vi "Process.vi"(8 "error in":errorcluster, 11 "Pump":refnum<class "Pump.lvclass">) -> (0 "error out":errorcluster, 3 "Pump out":refnum<class "Pump.lvclass">)   [LabVIEW 2014, in "Pump.lvclass"]
doc: "JKI State Machine Objects (SMO) 1.4.0.57\nJKI - JKI\nCopyright (c) 2018, JKI"
uses:
  Pump.lvclass
  <vilib>/JKI/JKI SMO/SMO/Typedefs/Parent Call--Enum.ctl
  Pump.lvclass/Pump.ctl
  Pump State - cluster.ctl
  <vilib>/addons/control/pid/pid.llb/PID Advanced (DBL).vi
  <vilib>/JKI/JKI SMO/SMO/SMO.lvclass
  <vilib>/addons/control/pid/NI_PID_pid.lvlib
panel:
  out "Pump State":T1(graph)
  # "For instructions on how to use the JKI State Machine Objects, examples and video tutorials, visit:\nhttp://jki.net/state-machine-objects/\n\nJKI State Machine Objects™\nhttp://jki.net/state-machine-objects/\nCopyright (C) 2005-2015, JKI <info@jki.net>\nALL RIGHTS RESERVED"
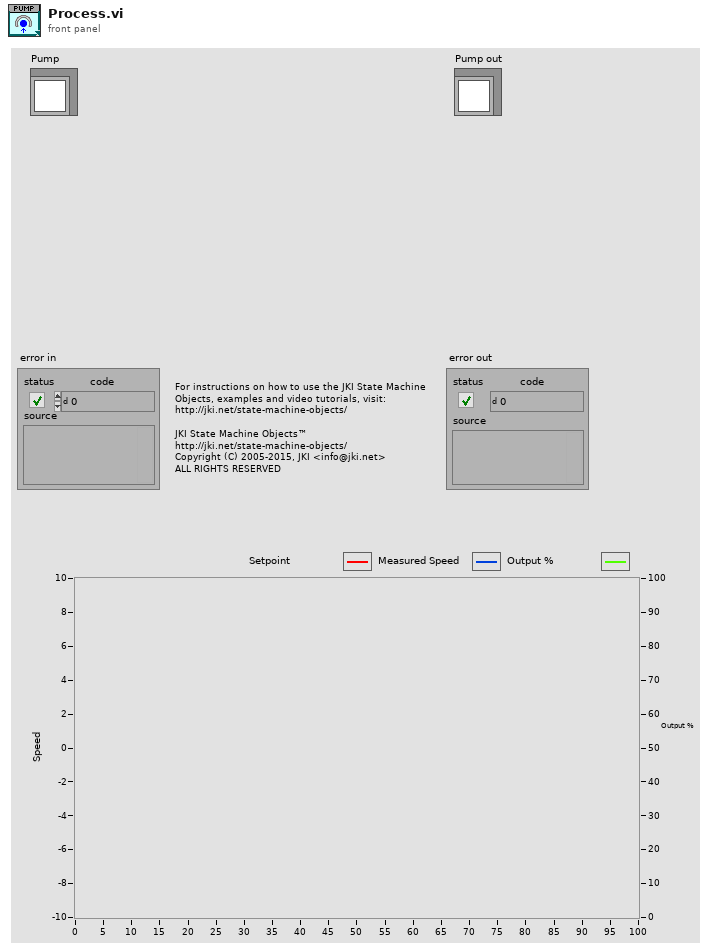
[diagram p1: front panel]
types:
  T1 = typedef "Pump.lvclass/Pump State - cluster.ctl" = cluster{"Pump Setpoint":dbl, "Pump Speed":dbl, "Output %":dbl}
  T2 = typedef "SMO.lvclass/Parent Call--Enum.ctl" = enum16{"Allows parent to run", "Does not request parent to run"}
  T3 = enum32{"invalid app kind", "Development System", "Run Time System", "Student Edition", "Embedded LabVIEW", "Evaluation", "Custom"}
  T4 = enum32{"Invalid", "Standard", "Closed", "Hidden", "Minimized", "Maximized"}
  T5 = cluster{"proportional gain (Kc)":dbl, "integral time (Ti, min)":dbl, "derivative time (Td, min)":dbl}
  T6 = typedef "Pump.lvclass/Parameters - cluster.ctl" = cluster{"Kc":dbl, "Ti":dbl, "Td":dbl, "Min Speed":dbl, "Max Speed":dbl}
  T7 = cluster{"Core":cluster{"Current VI Reference":refnum<vi>, "Close Panel on Exit?":bool, "error":errorcluster}, "Self Reference":refnum<class "Pump.lvclass">, "Parameters":T6, "Speed":dbl}
  T8 = cluster{"Current VI Reference":refnum<vi>, "Close Panel on Exit?":bool, "error":errorcluster}
  T9 = typedef "SMO.lvclass/Protected Events.ctl" = cluster{"StopProcesses":refnum<user-event>, "AbortProcesses":refnum<user-event>, "Config Changed":refnum<user-event>, "Dependency":refnum<user-event>}
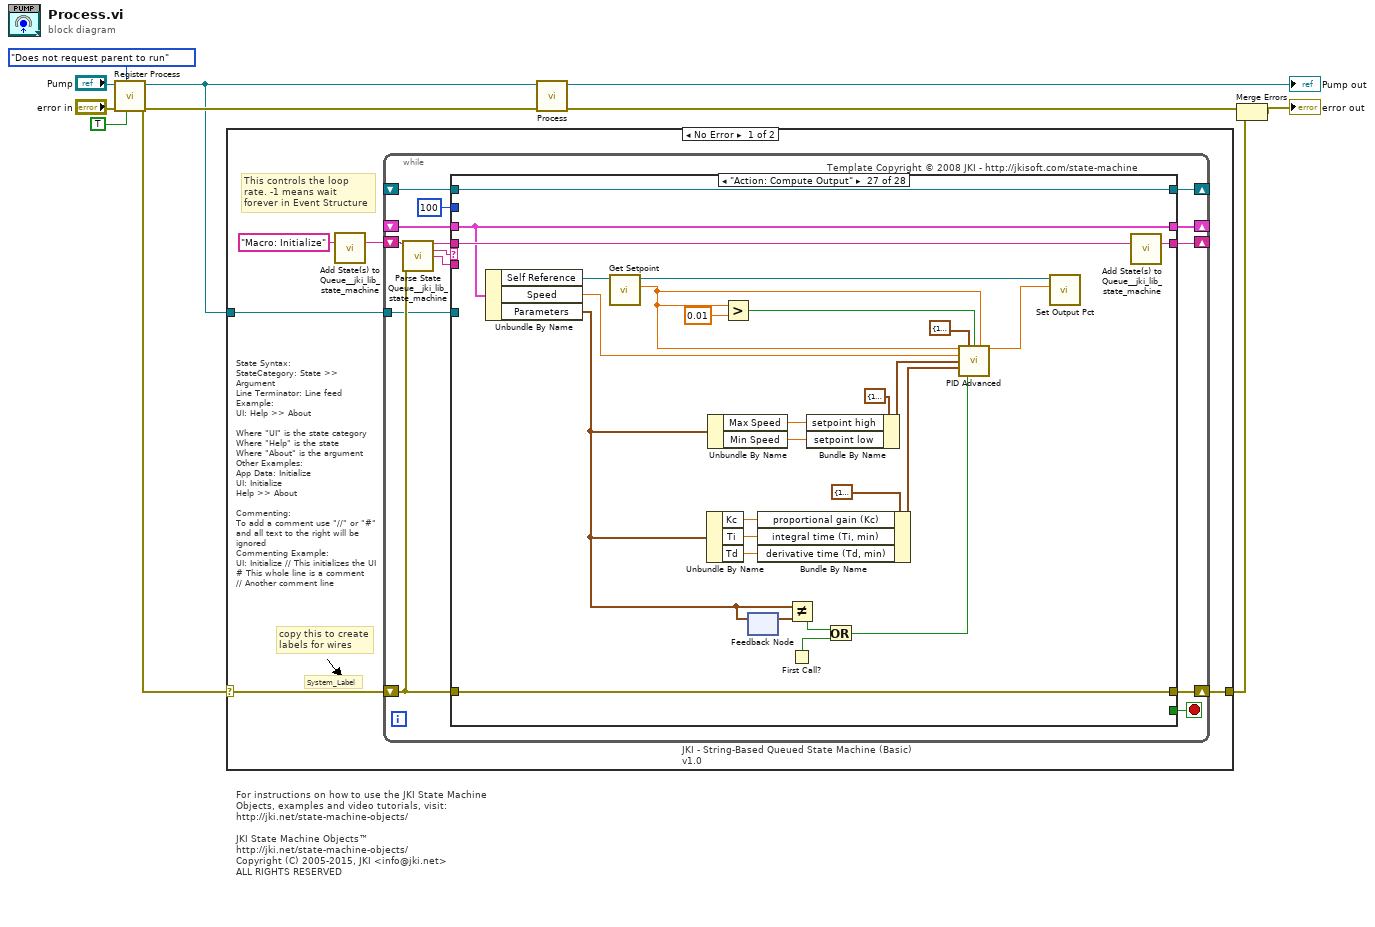
[diagram p0: block diagram]
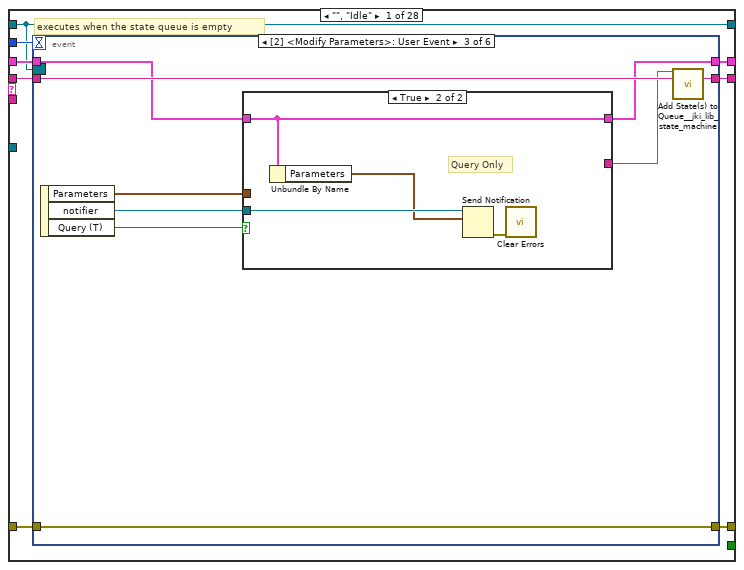
[diagram p2: hidden frame]
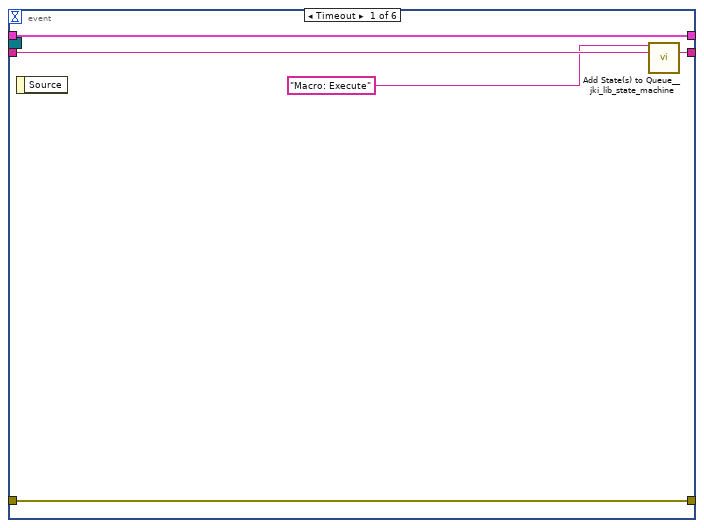
[diagram p3: hidden frame]
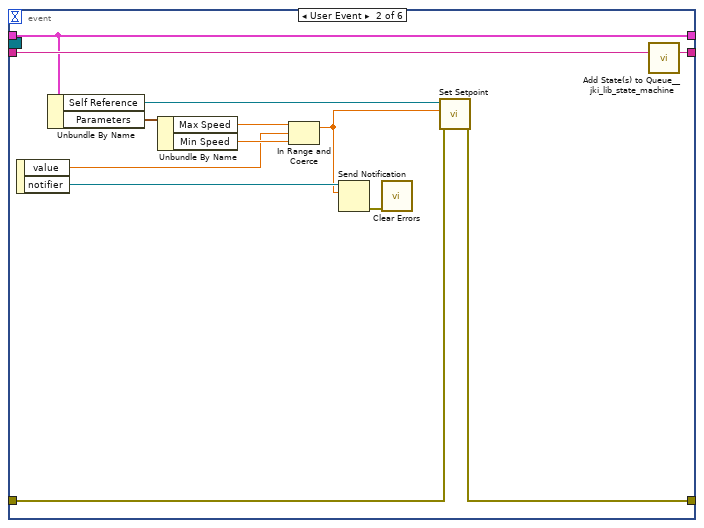
[diagram p4: hidden frame]
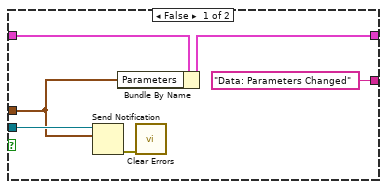
[diagram p5: hidden frame]
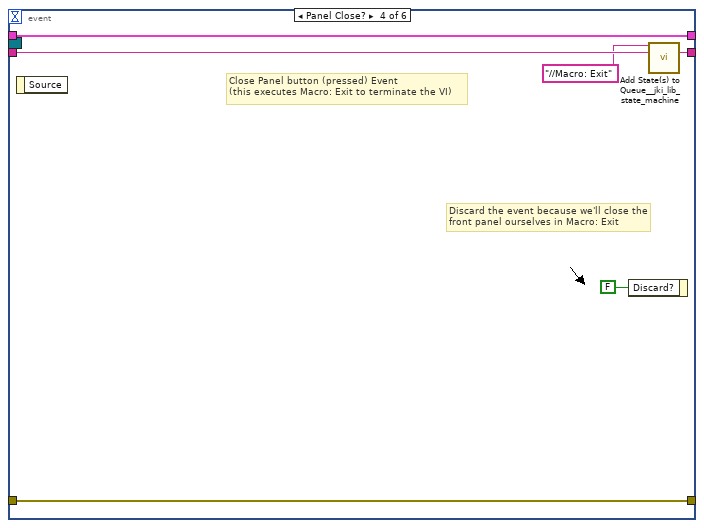
[diagram p6: hidden frame]
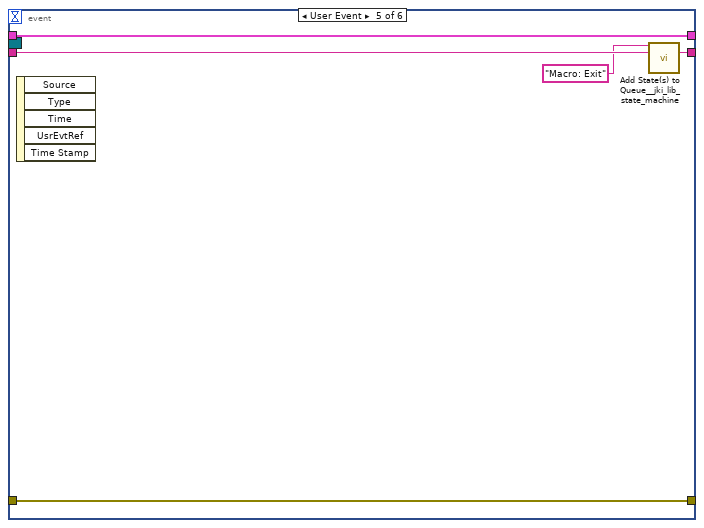
[diagram p7: hidden frame]
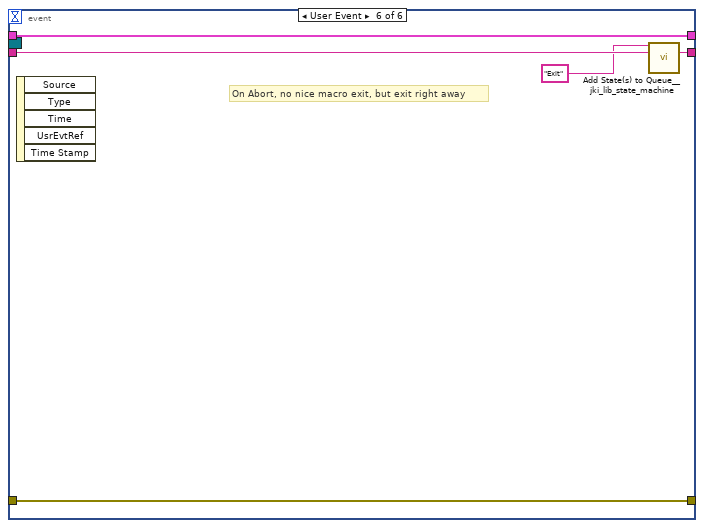
[diagram p8: hidden frame]
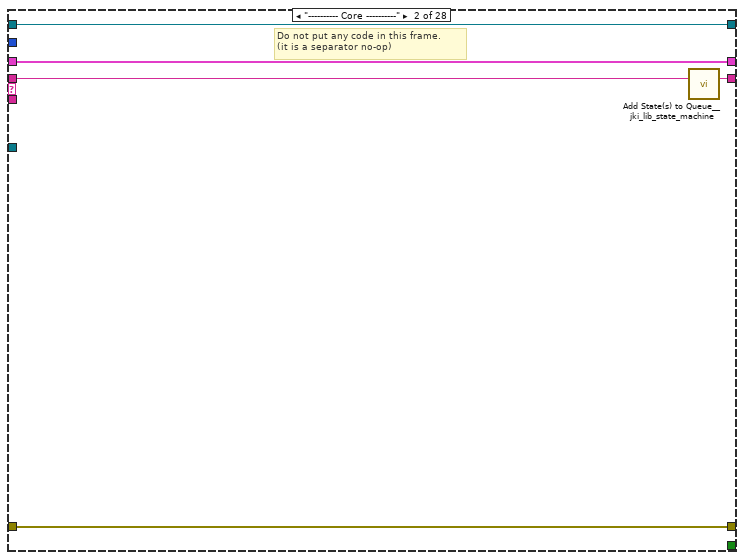
[diagram p9: hidden frame]
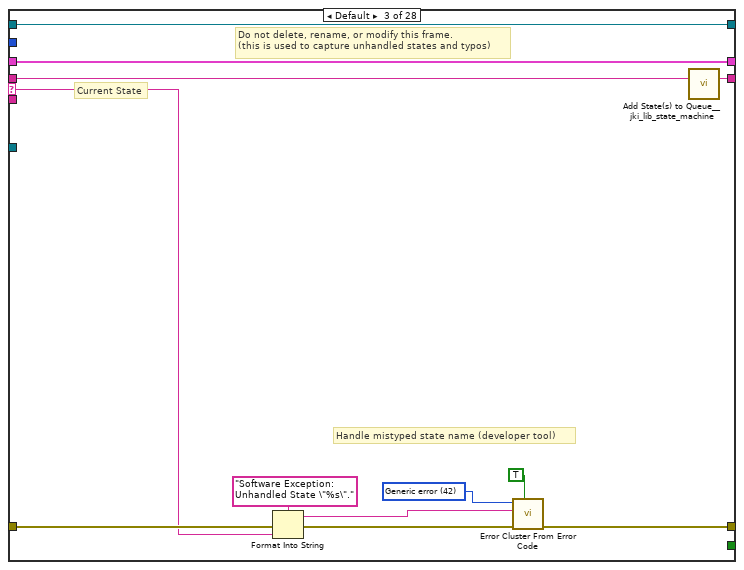
[diagram p10: hidden frame]
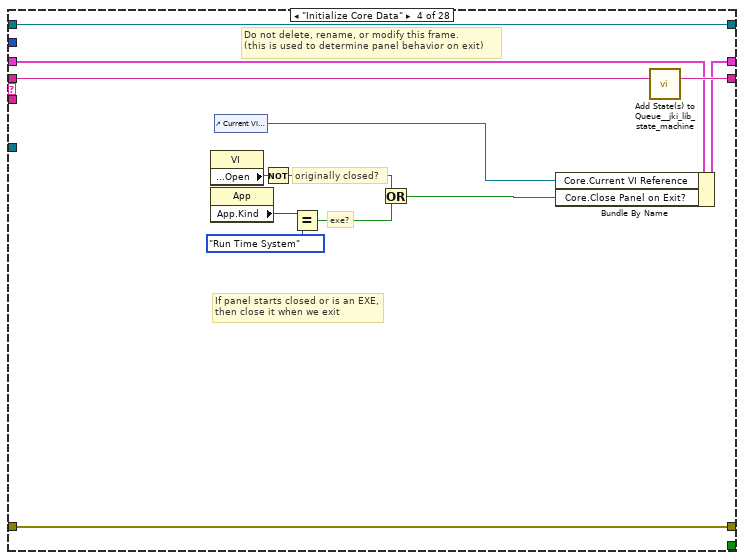
[diagram p11: hidden frame]
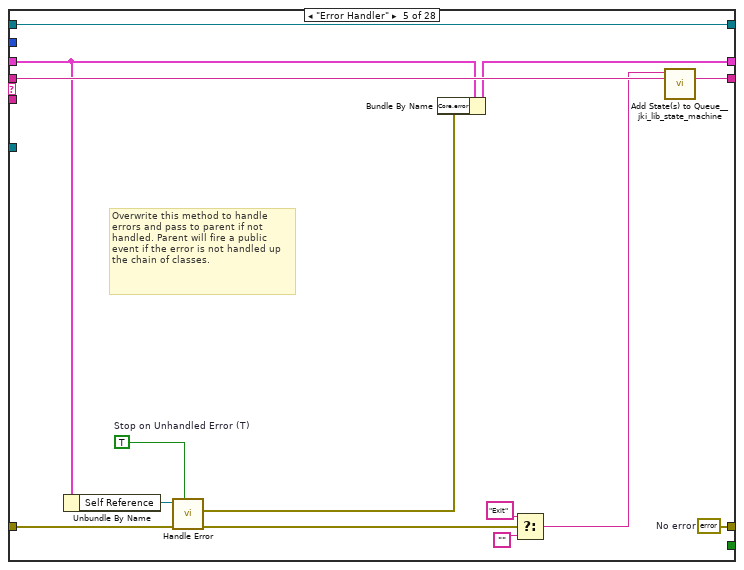
[diagram p12: hidden frame]
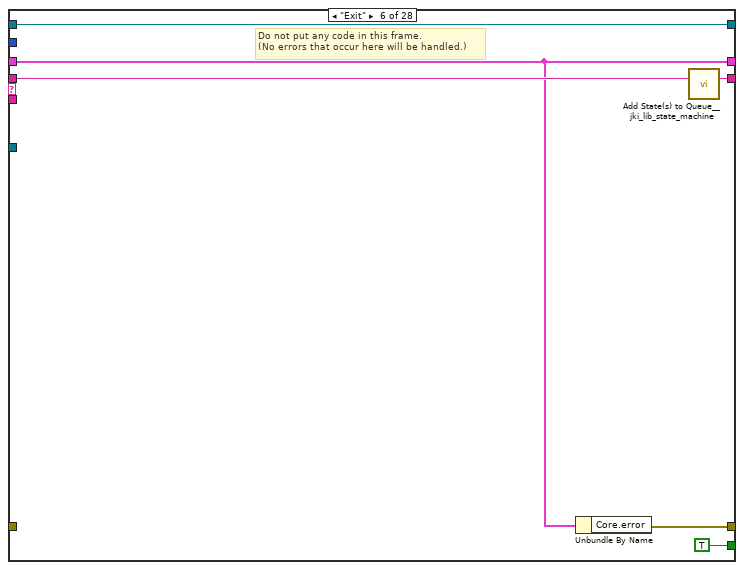
[diagram p13: hidden frame]
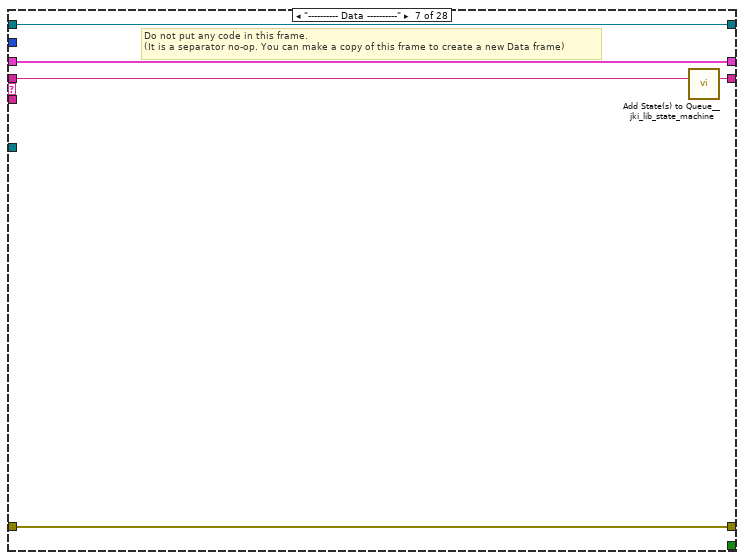
[diagram p14: hidden frame]
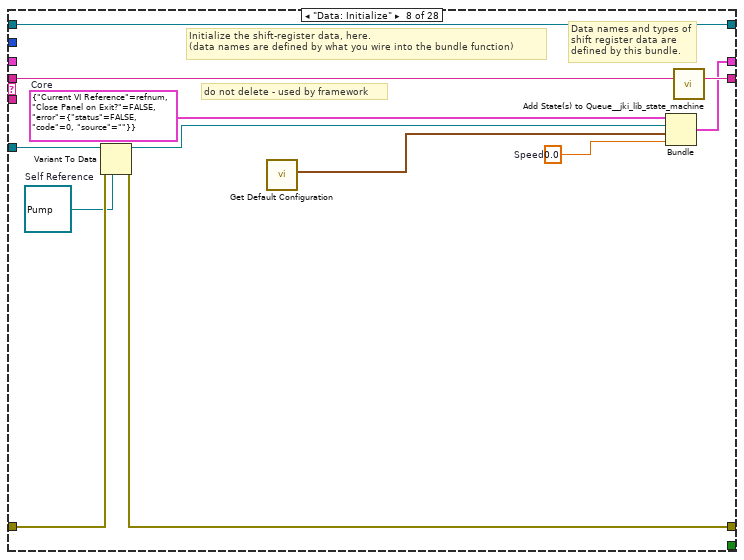
[diagram p15: hidden frame]
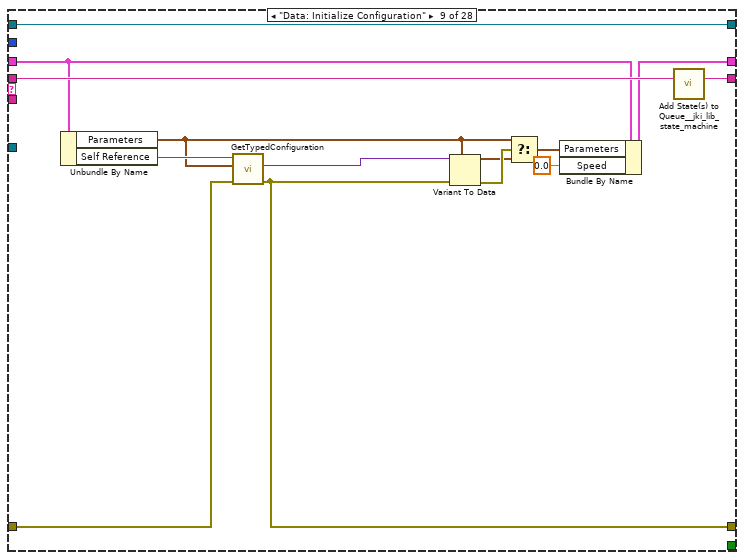
[diagram p16: hidden frame]
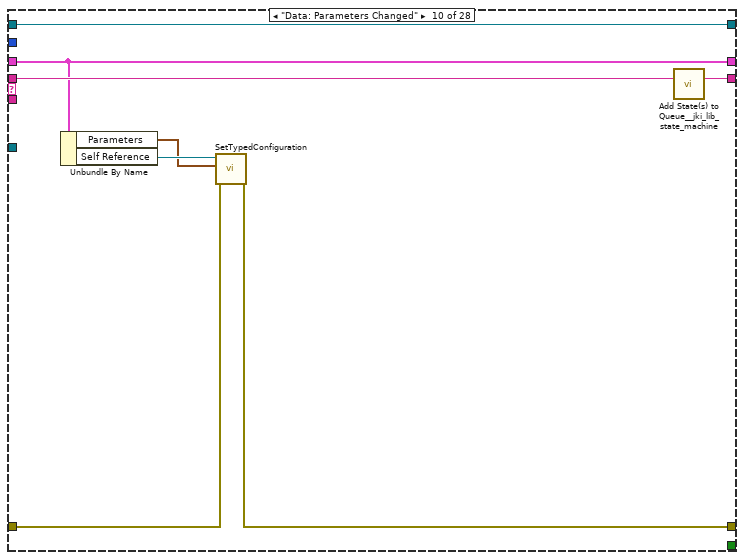
[diagram p17: hidden frame]
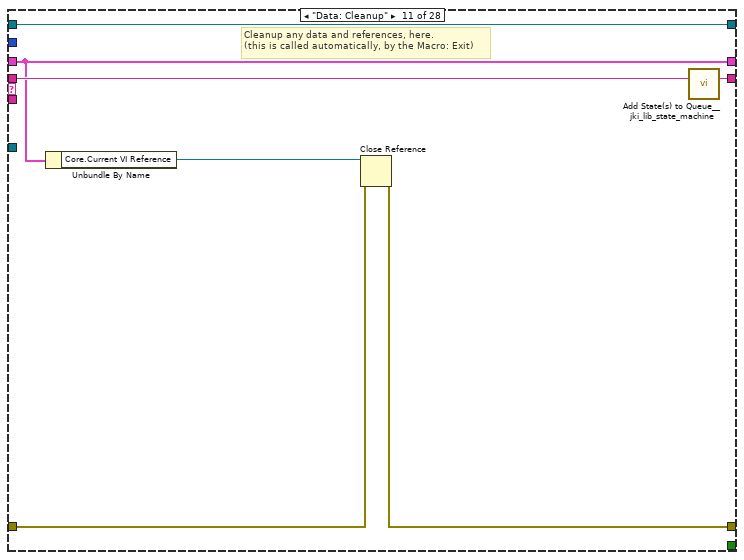
[diagram p18: hidden frame]
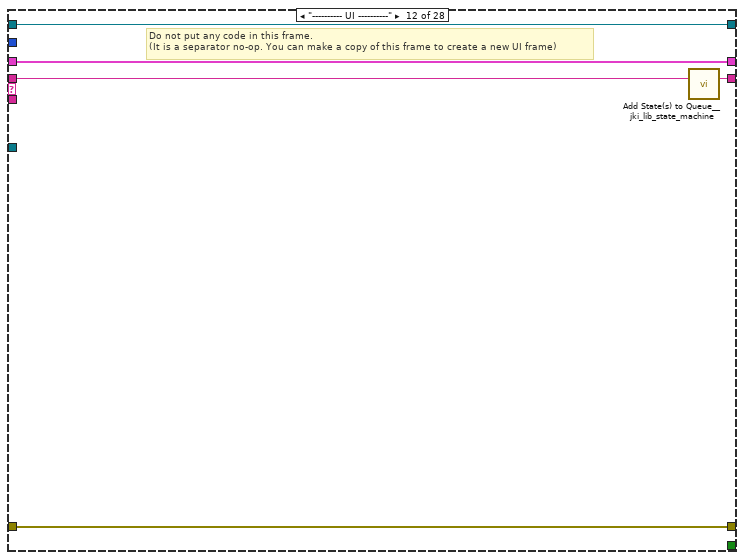
[diagram p19: hidden frame]
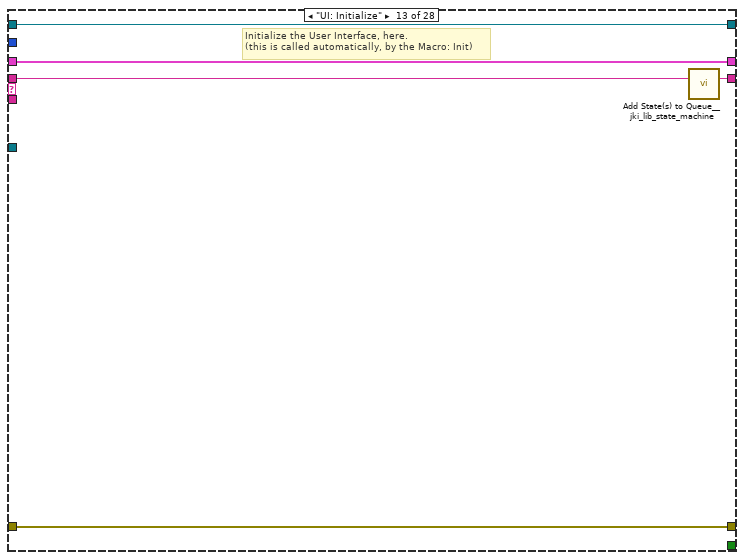
[diagram p20: hidden frame]
diagram:
  # "For instructions on how to use the JKI State Machine Objects, examples and video tutorials, visit:\nhttp://jki.net/state-machine-objects/\n\nJKI State Machine Objects™\nhttp://jki.net/state-machine-objects/\nCopyright (C) 2005-2015, JKI <info@jki.net>\nALL RIGHTS RESERVED"
  n1 = call <vilib>:"Register Process.vi"("Forces Self to Run (F)"=TRUE, "Parent Call"=Parent_Call--Enum."Does not request parent to run", "error in (no error)"="error in", "SMO"="Pump") -> ("error out"=w10:errorcluster, "SMO out"=w9:refnum<class "Pump.lvclass">)  [unwired: 6 in]
  n2 = case shown="No Error" w10 {
    selector: w10 -> [w12 w380]
    tunnel: w9 -> [w13 _]
    tunnel: [w11 w380] -> w7
    frame No Error {
      # "State Syntax:\nStateCategory: State >> Argument\nLine Terminator: Line feed\nExample:\nUI: Help >> About\n\nWhere \"UI\" is the state category\nWhere \"Help\" is the state\nWhere \"About\" is the argument\nOther Examples:\nApp Data: Initialize\nUI: Initialize\nHelp >> About\n\nCommenting:\nTo add a comment use \"//\" or \"#\" and all text to the right will be ignored\nCommenting Example:\nUI: Initialize // This initializes the UI\n# This whole line is a comment\n// Another comment line"
      # "copy this to create labels for wires"
      # "This controls the loop rate. -1 means wait forever in Event Structure"
      # "System_Label"
      n3 = call <vilib>:"Add State(s) to Queue__jki_lib_state_machine.vi"("State(s) in (\"\")"="Macro: Initialize") -> ("States Out"=w15:string)  [unwired: 14 in]
      n4 = while "JKI - String-Based Queued State Machine (Basic) v1.0" {
        shift-right: [w22] -> _
        shift-left: _ -> [w21]
        shift-right: [w25] -> w11
        shift-left: w12 -> [w19]
        shift-right: [w24] -> _
        shift-left: w15 -> [w26]
        tunnel: w13 -> [w18]
        shift-right: [w17] -> _
        shift-left: _ -> [w16]
        stop <- w23 stop-if-true
        # "Template Copyright © 2008 JKI - http://jkisoft.com/state-machine"
        n5 = call <vilib>:"Parse State Queue__jki_lib_state_machine.vi"("State Queue"=w26, "Error In (no error)"=w19) -> ("Remaining States"=w28:string, "Current State"=w29:string, "Arguments"=w27:string)  [unwired: 11 in]
        n6 = case shown="\"Action: Compute Output\"" w29 {
          selector: w29 -> [_ _ w97 _ _ _ _ _ _ _ _ _ _ _ _ _ _ _ _ _ _ _ _ _ _ _ _ _]
          tunnel: w28 -> [w37 w95 w101 w120 w134 w140 w145 w157 w171 w179 w186 w191 w196 w203 w219 w251 w260 w266 w280 w285 w296 w301 w313 w319 w324 w334 w361 w379]
          tunnel: w27 -> [_ _ _ _ _ _ _ _ _ _ _ _ _ w197 w213 _ _ _ _ _ _ _ _ _ _ _ _ _]
          tunnel: w21 -> [w35 w92 w99 w111 w128 w136 w142 _ w168 w172 w181 w188 w194 w201 w215 w248 w256 w262 w271 w282 w293 w298 w311 w317 w322 w331 w345 w376]
          tunnel: [w34 w93 w103 w117 w129 w135 w143 w153 w160 w174 w182 w189 w193 w198 w216 w249 w258 w264 w278 w283 w287 w299 w308 w315 w320 w330 w358 w369] -> w25
          tunnel: w19 -> [w33 w93 w102 w117 w130 _ w143 w154 w161 w175 w183 w189 w193 w199 w217 w249 w258 w264 w278 w283 w288 w299 w309 w315 w320 w326 w358 w370]
          tunnel: [w36 w94 w100 w119 w133 w139 w144 w156 w170 w178 w185 w190 w195 w202 w218 w250 w259 w265 w279 w284 w295 w300 w312 w318 w323 w333 w360 w378] -> w24
          tunnel: [_ _ _ _ _ TRUE _ _ _ _ _ _ _ _ _ _ _ _ _ _ _ _ _ _ _ _ _ _] -> w23
          tunnel: [w32 w92 w99 w118 w127 w136 w142 w155 w167 w172 w181 w188 w194 w201 w215 w248 w256 w262 w271 w282 w293 w298 w311 w317 w322 w331 w345 w375] -> w22
          tunnel: 100 ("Timeout") -> [w31 _ _ _ _ _ _ _ _ _ _ _ _ _ _ _ _ _ _ _ _ _ _ _ _ _ _ _]
          tunnel: w18 -> [_ _ _ _ _ _ _ w152 _ _ _ _ _ _ _ _ _ _ _ _ _ _ _ _ _ _ _ _]
          tunnel: [w30 w91 w96 w108 w132 w137 w141 w150 w169 w177 w180 w187 w192 w200 w212 w247 w257 w263 w272 w281 w294 w297 w302 w316 w321 w332 w359 w377] -> w17
          tunnel: w16 -> [w30 w91 w96 w108 w132 w137 w141 w150 w169 w177 w180 w187 w192 w200 w212 w247 w257 w263 w272 w281 w294 w297 _ w316 w321 w332 w359 w377]
          frame "", "Idle" {
            # "executes when the state queue is empty"
            n7 = event shown="[2] <Modify Parameters>: User Event" {
              selector: w30 -> [_ _ _ _ _ _]
              dyn-events: _ -> [_ _ _ _ _ _]
              timeout: w31 -> [_ _ _ _ _ _]
              tunnel: w37 -> [w42 w55 w64 w80 w85 w90]
              tunnel: [w41 w54 w63 w79 w84 w89] -> w36
              tunnel: w35 -> [w38 w45 w58 w77 w82 w87]
              tunnel: [w40 w43 w61 w78 w83 w88] -> w34
              tunnel: w33 -> [w40 w44 w61 w78 w83 w88]
              tunnel: [w38 w45 w57 w77 w82 w87] -> w32
              event Timeout {
                n8 = event-data() -> ()  [unwired: 1 in, 1 out]
                n9 = call <vilib>:"Add State(s) to Queue__jki_lib_state_machine.vi"("State(s) in Front (\"\")"="Macro: Execute", "State(s) in (\"\")"=w42) -> ("States Out"=w41:string)  [unwired: 13 in]
              }
              event User Event {
                n10 = event-data() -> ("value"=w48:dbl, "notifier"=w52:refnum<notifier>)  [unwired: 1 in]
                n11 = Unbundle By Name(w45) -> ("Self Reference"=w47:refnum<class "Pump.lvclass">, "Parameters"=w51:T6)
                n12 = Unbundle By Name(w51) -> ("Max Speed"=w50:dbl, "Min Speed"=w49:dbl)
                n13 = In Range and Coerce(upper limit=w50, x=w48, lower limit=w49) -> (coerced(x)=w46:dbl)  [unwired: 1 out]
                n14 = Send Notification(notification=w46, notifier=w52) -> (error out=w53:errorcluster)  [unwired: 1 in, 1 out]
                n15 = call <vilib>:"Clear Errors.vi"("error in (no error)"=w53) -> ()  [unwired: 5 in, 2 out]
                n16 = call "Set Setpoint.vi"("error in (no error)"=w44, "Setpoint"=w46, "Pump in"=w47) -> ("error out"=w43:errorcluster)  [unwired: 7 in, 1 out]
                n17 = call <vilib>:"Add State(s) to Queue__jki_lib_state_machine.vi"("State(s) in (\"\")"=w55) -> ("States Out"=w54:string)  [unwired: 14 in]
              }
              event User Event {
                n18 = event-data() -> ("Parameters"=w60:T6, "notifier"=w62:refnum<notifier>, "Query (T)"=w56:bool)  [unwired: 1 in]
                n19 = case shown="True" w56 {
                  tunnel: w62 -> [w69 w73]
                  tunnel: w60 -> [w68 _]
                  tunnel: ["Data: Parameters Changed" _] -> w59
                  tunnel: w58 -> [w66 w72]
                  tunnel: [w65 w72] -> w57
                  frame False {
                    n20 = Send Notification(notification=w68, notifier=w69) -> (error out=w70:errorcluster)  [unwired: 1 in, 1 out]
                    n21 = Bundle By Name(cluster=w66, "Parameters"=w68) -> (w65:T7)
                    n22 = call <vilib>:"Clear Errors.vi"("error in (no error)"=w70) -> ()  [unwired: 5 in, 2 out]
                  }
                  frame True {
                    # "Query Only"
                    n23 = Unbundle By Name(w72) -> ("Parameters"=w71:T6)
                    n24 = Send Notification(notification=w71, notifier=w73) -> (error out=w74:errorcluster)  [unwired: 1 in, 1 out]
                    n25 = call <vilib>:"Clear Errors.vi"("error in (no error)"=w74) -> ()  [unwired: 5 in, 2 out]
                  }
                }
                n26 = call <vilib>:"Add State(s) to Queue__jki_lib_state_machine.vi"("State(s) in Front (\"\")"=w59, "State(s) in (\"\")"=w64) -> ("States Out"=w63:string)  [unwired: 13 in]
              }
              event Panel Close? {
                # "Discard the event because we'll close the front panel ourselves in Macro: Exit"
                # "Close Panel button (pressed) Event\n(this executes Macro: Exit to terminate the VI)"
                n27 = event-data() -> ()  [unwired: 1 in, 1 out]
                n28 = event-data("Discard?"=FALSE) -> ()  [unwired: 1 in, 1 out]
                n29 = call <vilib>:"Add State(s) to Queue__jki_lib_state_machine.vi"("State(s) in Front (\"\")"="//Macro: Exit", "State(s) in (\"\")"=w80) -> ("States Out"=w79:string)  [unwired: 13 in]
              }
              event User Event {
                n30 = event-data() -> ()  [unwired: 1 in, 5 out]
                n31 = call <vilib>:"Add State(s) to Queue__jki_lib_state_machine.vi"("State(s) in Front (\"\")"="Macro: Exit", "State(s) in (\"\")"=w85) -> ("States Out"=w84:string)  [unwired: 13 in]
              }
              event User Event {
                # "On Abort, no nice macro exit, but exit right away"
                n32 = event-data() -> ()  [unwired: 1 in, 5 out]
                n33 = call <vilib>:"Add State(s) to Queue__jki_lib_state_machine.vi"("State(s) in Front (\"\")"="Exit", "State(s) in (\"\")"=w90) -> ("States Out"=w89:string)  [unwired: 13 in]
              }
            }
          }
          frame "---------- Core ----------" {
            # "Do not put any code in this frame.\n(it is a separator no-op)"
            n34 = call <vilib>:"Add State(s) to Queue__jki_lib_state_machine.vi"("State(s) in (\"\")"=w95) -> ("States Out"=w94:string)  [unwired: 14 in]
          }
          frame Default {
            w106 = 42 items=["No error", "Argument error", "Memory is full", "Out of zone", "End of file", "File already open", "Generic file I/O error", "File not found", "File permission error", "Disk is full", "Duplicate path", "Too many files open", "System feature not enabled", "Resource file not found", "Cannot add resource", "Resource not found", "Image not found", "Image memory error", "Pen does not exist", "Config type invalid", "Config token not found", "Config parse error", "Config memory error", "Bad external code format", "Bad external code offset", "External code not present", "Null window", "Destroy window error", "Null menu", "Print aborted", "Bad print record", "Print driver error", "Windows error during printing", "Memory error during printing", "Print dialog error", "Generic print error", "Invalid device refnum", "Device not found", "Device parameter error", "Device unit error", "Cannot open device", "Device call aborted", "Generic error", "Cancelled by user", "Object ID too low", "Object ID too high", "Object not in heap", "Unknown heap", "Unknown object (invalid DefProc)", "Unknown object (DefProc not in table)", "Message out of range", "Invalid (null) method", "Unknown message", "Manager call not supported", "Bad address", "Network operation in progress", "Network operation timed out", "Connection is busy", "Network attribute not supported", "Network error", "Address in use", "System out of memory", "Connection aborted", "Connection refused", "Not connected", "Already connected", "Connection closed", "Initialization error (interapplication manager)", "Bad occurrence", "Wait on unbound occurrence handler", "Occurrence queue overflow", "Datalog type conflict", "Unused", "Unrecognized type (interapplication manager)", "Memory corrupt", "Failed to make temporary DLL", "Old CIN version", "Drag socket not found", "Failed to load drop-object", "Failed to register OLE object", "Failed to release OLE object", "Format specifier type mismatch", "Unknown format specifier", "Too few format specifiers", "Too many format specifiers", "Scan failed", "Newer CIN version", "Error converting to variant", "Runtime menu error", "Password tampered", "Variant attribute not found", "Incompatible variant data type", "Event data is not available", "Event Store is not present", "Occurrence is not found", "Event Queue is not created", "Event info is not available", "Refnum passed is NULL", "Error retrieving Class GUID", "Error retrieving CoClass GUID", "Error retrieving TypeLib GUID.", "Bad built application magic bytes.", "Specific driver is different from the specific driver associated with the Logical Name.", "There is no session opened to the class driver.", "Max Error", "MAX - Error with config objects", "MAX - Error loading configuration", "MAX - Group not supported"]
            # "Current State"
            # "Do not delete, rename, or modify this frame.\n(this is used to capture unhandled states and typos)"
            # "Handle mistyped state name (developer tool)"
            n35 = Format Into String(format string="Software Exception: Unhandled State \"%s\"." ("message"), error in=w102, w97) -> (resulting string=w105:string, error out=w104:errorcluster)  [unwired: 1 in]
            n36 = call <vilib>:"Error Cluster From Error Code.vi"("show call chain? (False)"=TRUE, "error in (no error)"=w104, "error message (\"\")"=w105, "error code (0)"=w106) -> ("error out"=w103:errorcluster)  [unwired: 5 in]
            n37 = call <vilib>:"Add State(s) to Queue__jki_lib_state_machine.vi"("State(s) in (\"\")"=w101) -> ("States Out"=w100:string)  [unwired: 14 in]
          }
          frame "Initialize Core Data" {
            # "Do not delete, rename, or modify this frame.\n(this is used to determine panel behavior on exit)"
            # "originally closed?"
            # "exe?"
            # "If panel starts closed or is an EXE, then close it when we exit"
            n38 = property class="VI"() -> ("Front Panel.Open"=w116:bool)  [unwired: 2 in, 2 out]
            n39 = property class="App"() -> ("App.Kind"=w115:T3)  [unwired: 2 in, 2 out]
            n40 = control-ref of="Current VI Reference"() -> (w109:refnum<vi>)
            n41 = Not(x=w116) -> (.not. x?=w113:bool)
            n42 = Equal?(x=w115, y=T3."Run Time System" ("Application:Kind")) -> (x = y?=w112:bool)
            n43 = Or(x=w113, y=w112) -> (x .or. y?=w110:bool)
            n44 = Bundle By Name(cluster=w111, "Core.Current VI Reference"=w109, "Core.Close Panel on Exit?"=w110) -> (w118:T7)
            n45 = call <vilib>:"Add State(s) to Queue__jki_lib_state_machine.vi"("State(s) in (\"\")"=w120) -> ("States Out"=w119:string)  [unwired: 14 in]
          }
          frame "Error Handler" {
            w121 = TRUE  # Stop on Unhandled Error (T)
            w129 = errorcluster {"status"=FALSE, "code"=0, "source"=""}  # No error
            # "Overwrite this method to handle errors and pass to parent if not handled. Parent will fire a public event if the error is not handled up the chain of classes."
            n46 = Unbundle By Name(w128) -> ("Self Reference"=w131:refnum<class "Pump.lvclass">)
            n47 = call-dynamic "Handle Error.vi"("Stop on Unhandled Error (T)"=w121, "error in"=w130, "SMO"=w131) -> ("handling error"=w122:errorcluster, "Unhandled error"=w125:errorcluster)  [unwired: 6 in, 1 out]
            n48 = Bundle By Name(cluster=w128, "Core.error"=w125) -> (w127:T7)
            n49 = Select(t="Exit", s=w122, f="") -> (s? t:f=w126:string)
            n50 = call <vilib>:"Add State(s) to Queue__jki_lib_state_machine.vi"("State(s) in Front (\"\")"=w126, "State(s) in (\"\")"=w134) -> ("States Out"=w133:string)  [unwired: 13 in]
          }
          frame "Exit" {
            # "Do not put any code in this frame.\n(No errors that occur here will be handled.)"
            n51 = Unbundle By Name(w136) -> ("Core.error"=w135:errorcluster)
            n52 = call <vilib>:"Add State(s) to Queue__jki_lib_state_machine.vi"("State(s) in (\"\")"=w140) -> ("States Out"=w139:string)  [unwired: 14 in]
          }
          frame "---------- Data ----------" {
            # "Do not put any code in this frame.\n(It is a separator no-op. You can make a copy of this frame to create a new Data frame)"
            n53 = call <vilib>:"Add State(s) to Queue__jki_lib_state_machine.vi"("State(s) in (\"\")"=w145) -> ("States Out"=w144:string)  [unwired: 14 in]
          }
          frame "Data: Initialize" {
            w146 = 0.0  # Speed
            w148 = refnum<class "Pump.lvclass"> refnum  # Self Reference
            w149 = T8 {"Current VI Reference"=refnum, "Close Panel on Exit?"=FALSE, "error"={"status"=FALSE, "code"=0, "source"=""}}  # Core
            # "do not delete - used by framework"
            # "Data names and types of shift register data are defined by this bundle."
            # "Initialize the shift-register data, here.\n(data names are defined by what you wire into the bundle function)"
            n54 = Variant To Data(error in=w154, type=w148, Variant=w152) -> (data=w151:refnum<class "Pump.lvclass">, error out=w153:errorcluster)
            n55 = call "Get Default Configuration.vi"() -> ("Parameters"=w147:T6)  [unwired: 11 in]
            n56 = Bundle("Core"=w149, "Self Reference"=w151, "Parameters"=w147, "Speed"=w146) -> (w155:T7)  [unwired: 1 in]
            n57 = call <vilib>:"Add State(s) to Queue__jki_lib_state_machine.vi"("State(s) in (\"\")"=w157) -> ("States Out"=w156:string)  [unwired: 14 in]
          }
          frame "Data: Initialize Configuration" {
            n58 = Unbundle By Name(w168) -> ("Parameters"=w159:T6, "Self Reference"=w163:refnum<class "Pump.lvclass">)
            n59 = call <vilib>:"GetTypedConfiguration.vi"("error in (no error)"=w161, "Default value"=w159, "SMO"=w163) -> ("error out"=w160:errorcluster, "Variant"=w162:variant)  [unwired: 4 in, 3 out]
            n60 = Variant To Data(error in=w160, type=w159, Variant=w162) -> (data=w165:T6, error out=w166:errorcluster)
            n61 = Select(t=w159, s=w166, f=w165) -> (s? t:f=w164:T6)
            n62 = Bundle By Name(cluster=w168, "Parameters"=w164, "Speed"=0.0 ("Setpoint")) -> (w167:T7)
            n63 = call <vilib>:"Add State(s) to Queue__jki_lib_state_machine.vi"("State(s) in (\"\")"=w171) -> ("States Out"=w170:string)  [unwired: 14 in]
          }
          frame "Data: Parameters Changed" {
            n64 = Unbundle By Name(w172) -> ("Parameters"=w173:T6, "Self Reference"=w176:refnum<class "Pump.lvclass">)
            n65 = call <vilib>:"SetTypedConfiguration.vi"("error in (no error)"=w175, "Default value"=w173, "SMO"=w176) -> ("error out"=w174:errorcluster)  [unwired: 6 in, 2 out]
            n66 = call <vilib>:"Add State(s) to Queue__jki_lib_state_machine.vi"("State(s) in (\"\")"=w179) -> ("States Out"=w178:string)  [unwired: 14 in]
          }
          frame "Data: Cleanup" {
            # "Cleanup any data and references, here.\n(this is called automatically, by the Macro: Exit)"
            n67 = Unbundle By Name(w181) -> ("Core.Current VI Reference"=w184:refnum<vi>)
            n68 = Close Reference(reference=w184, error in (no error)=w183) -> (error out=w182:errorcluster)
            n69 = call <vilib>:"Add State(s) to Queue__jki_lib_state_machine.vi"("State(s) in (\"\")"=w186) -> ("States Out"=w185:string)  [unwired: 14 in]
          }
          frame "---------- UI ----------" {
            # "Do not put any code in this frame.\n(It is a separator no-op. You can make a copy of this frame to create a new UI frame)"
            n70 = call <vilib>:"Add State(s) to Queue__jki_lib_state_machine.vi"("State(s) in (\"\")"=w191) -> ("States Out"=w190:string)  [unwired: 14 in]
          }
          frame "UI: Initialize" {
            # "Initialize the User Interface, here.\n(this is called automatically, by the Macro: Init)"
            n71 = call <vilib>:"Add State(s) to Queue__jki_lib_state_machine.vi"("State(s) in (\"\")"=w196) -> ("States Out"=w195:string)  [unwired: 14 in]
          }
          frame "UI: Cursor Set" {
            # "Argument"
            # "Initialize the User Interface, here.\n(this is called automatically, by the Macro: Init)"
            n72 = disable-structure shown="Default" {
              disable-tunnel: w199 -> [w204 w207]
              disable-tunnel: [w204 w206] -> w198
              disable-tunnel: w197 -> [_ w205]
              frame condition #0 {
              }
              frame condition #1 (active) {
                n73 = case shown="\"Idle\", Default" w205 {
                  tunnel: w207 -> [w209 w211]
                  tunnel: [w208 w210] -> w206
                  frame "Idle", Default {
                    n74 = call <vilib>:"Unset Busy.vi"("error in (no error)"=w209) -> ("error out"=w208:errorcluster)  [unwired: 10 in]
                  }
                  frame "Busy" {
                    n75 = call <vilib>:"Set Busy.vi"("error in (no error)"=w211) -> ("error out"=w210:errorcluster)  [unwired: 9 in, 1 out]
                  }
                }
              }
            }
            n76 = call <vilib>:"Add State(s) to Queue__jki_lib_state_machine.vi"("State(s) in (\"\")"=w203) -> ("States Out"=w202:string)  [unwired: 14 in]
          }
          frame "UI: Front Panel State" {
            # "Argument"
            # "Set Front Panel Open or Closed\n(Usage: \"UI: Front Panel State >> Open|Close\")"
            n77 = Unbundle By Name(w215) -> ("Core.Current VI Reference"=w214:refnum<vi>)
            n78 = disable-structure shown="Default" {
              disable-tunnel: w217 -> [w223 w246]
              disable-tunnel: [w222 w246] -> w216
              disable-tunnel: w214 -> [w221 _]
              disable-tunnel: w213 -> [w220 _]
              frame condition #0 (active) {
                n79 = case shown="\"Close\"" w220 {
                  tunnel: w223 -> [w227 w240]
                  tunnel: [w229 w241] -> w222
                  tunnel: w221 -> [w228 w238]
                  frame "Open", Default {
                    n80 = property class="VI"(reference=w228, error in=w227) -> (reference out=w225:refnum<vi>, error out=w226:errorcluster, "FP.State"=w224:T4)
                    n81 = case shown="\"Closed\"" w224 {
                      tunnel: [w232 w235] -> w229
                      tunnel: w226 -> [w231 w235]
                      tunnel: w225 -> [w230 _]
                      frame "Closed" {
                        n82 = invoke class="VI" method="FP.Open"(reference=w230, error in=w231, "Activate"=TRUE, "State"=T4."Standard") -> (error out=w232:errorcluster)  [unwired: 1 in, 4 out]
                      }
                      frame Default {
                      }
                    }
                  }
                  frame "Close" {
                    n83 = property class="VI"(reference=w238, error in=w240) -> (reference out=w237:refnum<vi>, error out=w239:errorcluster, "FP.State"=w236:T4)
                    n84 = case shown="Default" w236 {
                      tunnel: [w242 w245] -> w241
                      tunnel: w239 -> [w242 w244]
                      tunnel: w237 -> [_ w243]
                      frame "Invalid", "Closed" {
                      }
                      frame Default {
                        n85 = invoke class="VI" method="FP.Close"(reference=w243, error in=w244) -> (error out=w245:errorcluster)  [unwired: 1 in, 2 out]
                      }
                    }
                  }
                }
              }
              frame condition #1 {
              }
            }
            n86 = call <vilib>:"Add State(s) to Queue__jki_lib_state_machine.vi"("State(s) in (\"\")"=w219) -> ("States Out"=w218:string)  [unwired: 14 in]
          }
          frame "---------- Macro ----------" {
            # "Do not put any code in this frame.\n(It is a separator no-op. You can make a copy of this frame to create a new Macro frame)"
            n87 = call <vilib>:"Add State(s) to Queue__jki_lib_state_machine.vi"("State(s) in (\"\")"=w251) -> ("States Out"=w250:string)  [unwired: 14 in]
          }
          frame "Macro: Initialize" {
            w254 = "//UI: Initialize\n//UI: Front Panel State >> Open"  # //UI: Initialize //UI: Front Panel State >> Open
            # "Initialization Macro\n(This is called once, when the VI starts)"
            n88 = call <vilib>:"Add State(s) to Queue__jki_lib_state_machine.vi"("State(s) in Front (\"\")"="Data: Initialize\nInitialize Core Data\nEvents: Register\nData: Initialize Configuration", "State(s) in (\"\")"="Process: Sync", "State(s) at Back (\"\")"=w254) -> ("States Out"=w253:string)  [unwired: 12 in]
            n89 = call <vilib>:"Add State(s) to Queue__jki_lib_state_machine.vi"("State(s) in Front (\"\")"=w253, "State(s) in (\"\")"=w260) -> ("States Out"=w259:string)  [unwired: 13 in]
          }
          frame "Macro: Execute" {
            n90 = call <vilib>:"Add State(s) to Queue__jki_lib_state_machine.vi"("State(s) in Front (\"\")"="Action: Read Speed\nAction: Compute Output\nAction: Control Pump", "State(s) in (\"\")"=w266) -> ("States Out"=w265:string)  [unwired: 13 in]
          }
          frame "Macro: Exit" {
            # "Exit Macro\n(This is called once, when the VI exits)"
            n91 = Unbundle By Name(w271) -> ("Core.Close Panel on Exit?"=w277:bool)
            n92 = Select(t="UI: Front Panel State >> Close", s=w277, f="") -> (s? t:f=w274:string)
            n93 = call <vilib>:"Add State(s) to Queue__jki_lib_state_machine.vi"("State(s) in Front (\"\")"="Data: Cleanup\nEvents: Unregister", "State(s) in (\"\")"="Process: Sync", "State(s) at Back (\"\")"="Exit") -> ("States Out"=w268:string)  [unwired: 12 in]
            n94 = call <vilib>:"Add State(s) to Queue__jki_lib_state_machine.vi"("State(s) in (\"\")"=w274, "State(s) at Back (\"\")"=w268) -> ("States Out"=w273:string)  [unwired: 13 in]
            n95 = call <vilib>:"Add State(s) to Queue__jki_lib_state_machine.vi"("State(s) in Front (\"\")"=w273, "State(s) in (\"\")"=w280) -> ("States Out"=w279:string)  [unwired: 13 in]
          }
          frame "---------- Process ----------" {
            # "Template Separator\n(You can make a copy of, or modify, this frame)"
            n96 = call <vilib>:"Add State(s) to Queue__jki_lib_state_machine.vi"("State(s) in (\"\")"=w285) -> ("States Out"=w284:string)  [unwired: 14 in]
          }
          frame "Process: Sync" {
            n97 = Unbundle By Name(w293) -> ("Self Reference"=w289:refnum<class "Pump.lvclass">)
            n98 = call <vilib>:"WaitOnProcessSync.vi"("error in (no error)"=w288, "SMO"=w289) -> ("error out"=w287:errorcluster, "Don't run?"=w292:bool)  [unwired: 7 in, 1 out]
            n99 = Select(t="Data: Cleanup\nEvents: Unregister\nExit", s=w292, f="") -> (s? t:f=w286:string)
            n100 = call <vilib>:"Add State(s) to Queue__jki_lib_state_machine.vi"("State(s) in Front (\"\")"=w286, "State(s) in (\"\")"=w296) -> ("States Out"=w295:string)  [unwired: 13 in]
          }
          frame "---------- Events ----------" {
            # "Template Separator\n(You can make a copy of, or modify, this frame)"
            n101 = call <vilib>:"Add State(s) to Queue__jki_lib_state_machine.vi"("State(s) in (\"\")"=w301) -> ("States Out"=w300:string)  [unwired: 14 in]
          }
          frame "Events: Register" {
            # "Expand to add\nmore events"
            n102 = Unbundle By Name(w311) -> ("Self Reference"=w305:refnum<class "Pump.lvclass">)
            n103 = call <vilib>:"GetProtectedEvents.vi"("SMO"=w305) -> ("error out"=w306:errorcluster, "SMO Protected Events"=w310:T9)  [unwired: 8 in, 1 out]
            n104 = Unbundle By Name(w305) -> ("Query Event"=w304:refnum<user-event>, "Modify Parameters"=w303:refnum<user-event>)
            n105 = register-events(w310, w304, w303) -> (reference out=w302:refnum<event-registration>, error out=w307:errorcluster)  [unwired: 2 in]
            n106 = Merge Errors(w309, w307, w306) -> (w308:errorcluster)
            n107 = call <vilib>:"Add State(s) to Queue__jki_lib_state_machine.vi"("State(s) in (\"\")"=w313) -> ("States Out"=w312:string)  [unwired: 14 in]
          }
          frame "Events: Unregister" {
            n108 = Unregister For Events(event registration refnum=w316, error in=w315) -> (error out=w314:errorcluster)
            n109 = call <vilib>:"Clear Errors.vi"("error in (no error)"=w314) -> ()  [unwired: 5 in, 2 out]
            n110 = call <vilib>:"Add State(s) to Queue__jki_lib_state_machine.vi"("State(s) in (\"\")"=w319) -> ("States Out"=w318:string)  [unwired: 14 in]
          }
          frame "---------- Action ----------" {
            n111 = call <vilib>:"Add State(s) to Queue__jki_lib_state_machine.vi"("State(s) in (\"\")"=w324) -> ("States Out"=w323:string)  [unwired: 14 in]
          }
          frame "Action: Control Pump" {
            n112 = Unbundle By Name(w331) -> ("Self Reference"=w329:refnum<class "Pump.lvclass">)
            n113 = call-dynamic "Get Output Pct.vi"("error in (no error)"=w326, "Pump in"=w329) -> ("error out"=w325:errorcluster, "Output %"=w327:dbl, "Pump out"=w328:refnum<class "Pump.lvclass">)  [unwired: 7 in]
            n114 = call-dynamic "writePumpSpeed.vi"("error in (no error)"=w325, "Output %"=w327, "Pump in"=w328) -> ("error out"=w330:errorcluster)  [unwired: 7 in, 1 out]
            n115 = call <vilib>:"Add State(s) to Queue__jki_lib_state_machine.vi"("State(s) in (\"\")"=w334) -> ("States Out"=w333:string)  [unwired: 14 in]
          }
          frame "Action: Compute Output" {
            n116 = Unbundle By Name(w345) -> ("Self Reference"=w357:refnum<class "Pump.lvclass">, "Speed"=w356:dbl, "Parameters"=w340:T6)
            n117 = call "Get Setpoint.vi"("Pump in"=w357) -> ("Pump Setpoint"=w338:dbl, "Pump out"=w347:refnum<class "Pump.lvclass">)  [unwired: 8 in, 1 out]
            n118 = Unbundle By Name(w340) -> ("Kc"=w350:dbl, "Ti"=w349:dbl, "Td"=w348:dbl)
            n119 = Unbundle By Name(w340) -> ("Max Speed"=w342:dbl, "Min Speed"=w343:dbl)
            n120 = Greater?(x=w338, y=0.01) -> (0:w339:bool)
            n121 = feedback #1() -> (w354:T6)  [unwired: 1 in]
            n122 = feedback-in #1(w340) -> ()
            n123 = Bundle By Name(cluster=T5 {"proportional gain (Kc)"=1.0, "integral time (Ti, min)"=0.01, "derivative time (Td, min)"=0.0} ("PID gains"), "proportional gain (Kc)"=w350, "integral time (Ti, min)"=w349, "derivative time (Td, min)"=w348) -> (w351:T5)
            n124 = Not Equal?(x=w340, y=w354) -> (x != y?=w353:bool)
            n125 = First Call?() -> (First Call?: T/F=w336:bool)
            n126 = Bundle By Name(cluster=cluster{"setpoint high":dbl, "setpoint low":dbl} {"setpoint high"=100.0, "setpoint low"=0.0} ("setpoint range"), "setpoint high"=w342, "setpoint low"=w343) -> (w337:cluster{"setpoint high":dbl, "setpoint low":dbl})
            n127 = Or(x=w353, y=w336) -> (x .or. y?=w335:bool)
            n128 = call-poly <vilib>:"PID Advanced.vi"("setpoint"=w338, "output range"=cluster{"output high":dbl, "output low":dbl} {"output high"=100.0, "output low"=0.0}, "auto? (T)"=w339, "manual control"=w338, "process variable"=w356, "setpoint range"=w337, "PID gains"=w351, "reinitialize? (F)"=w335) -> ("output"=w346:dbl)  [unwired: 6 in, 1 out]
            n129 = call "Set Output Pct.vi"("Output %"=w346, "Pump in"=w347) -> ()  [unwired: 8 in, 2 out]
            n130 = call <vilib>:"Add State(s) to Queue__jki_lib_state_machine.vi"("State(s) in (\"\")"=w361) -> ("States Out"=w360:string)  [unwired: 14 in]
          }
          frame "Action: Read Speed" {
            n131 = Unbundle By Name(w376) -> ("Self Reference"=w364:refnum<class "Pump.lvclass">)
            n132 = call-dynamic "readPumpSpeed.vi"("Pump in"=w364) -> ("error out"=w372:errorcluster, "Pump Speed"=w373:dbl, "Pump out"=w367:refnum<class "Pump.lvclass">)  [unwired: 8 in]
            n133 = call-dynamic "Get Output Pct.vi"("Pump in"=w364) -> ("error out"=w362:errorcluster, "Output %"=w363:dbl)  [unwired: 8 in, 1 out]
            n134 = call "Get Setpoint.vi"("Pump in"=w364) -> ("error out"=w371:errorcluster, "Pump Setpoint"=w374:dbl)  [unwired: 8 in, 1 out]
            n135 = Bundle By Name(cluster=w376, "Speed"=w373) -> (w375:T7)
            n136 = Bundle(cluster=T1 {"Pump Setpoint"=0.0, "Pump Speed"=0.0, "Output %"=0.0} ("Pump State"), "Pump Setpoint"=w374, "Pump Speed"=w373, "Output %"=w363) -> (w366:T1)
            "Pump State" <- w366
            n137 = call "Generate Pump State Event.vi"("Pump State"=w366, "Pump in"=w367) -> ("error out"=w365:errorcluster)  [unwired: 8 in, 1 out]
            n138 = Merge Errors(w370, w372, w371, w365, w362) -> (w369:errorcluster)
            n139 = call <vilib>:"Add State(s) to Queue__jki_lib_state_machine.vi"("State(s) in (\"\")"=w379) -> ("States Out"=w378:string)  [unwired: 14 in]
          }
        }
      }
    }
    frame Error {
    }
  }
  n140 = call-parent "Process.vi"("error in"=w10, "SMO"=w9) -> ("error out"=w8:errorcluster, "SMO out"=→"Pump out":refnum<class "Pump.lvclass">)  [unwired: 8 in]
  n141 = Merge Errors(w8, w7) -> (→"error out":errorcluster)
